vi "[ex ce] 1 Simplest client example.vi"() -> ()   [LabVIEW 2021]
doc: "<B>Simplest client example</B>\n\nThis example demonstrates simplest method to use CalcExpress for remote computation.\n\nTo execute this example, you need run <B>[ex ce] CE Server Example.vi</B> on either local or remote computer.\n\n::: CalcExpress Toolkit :::\nCopyright (c) 2000-2026 Konstantin Shifershteyn. All rights reserved."
uses:
  vi.lib/addons/CalcExpress/cetypes.llb/CalcExpress Data Type.ctl
panel:
  in  "Comment":string="To execute this example, you need run the \"[ex ce] CE Server Example.vi\" on either local or remote computer.\n---------------------------\nThis example demonstrates simplest method to use CalcExpress for remote computation.\n"
  in  "use TCP for local":bool
  in  "expression":string="/* initializes array of values in the range from -6*pi to 6*pi with step equal to 5 radians */\nx = nvecifs(-pi(6),pi(6), rad(5));\n\nsinc(x)  /* computes sin(x)/x */"
  out "graph":dbl[](graph)
  out "value type":T1=enum."DBL Number"
  out "error out":errorcluster
  in  "port":u32=3363
  in  "machine name (empty - localhost)":string
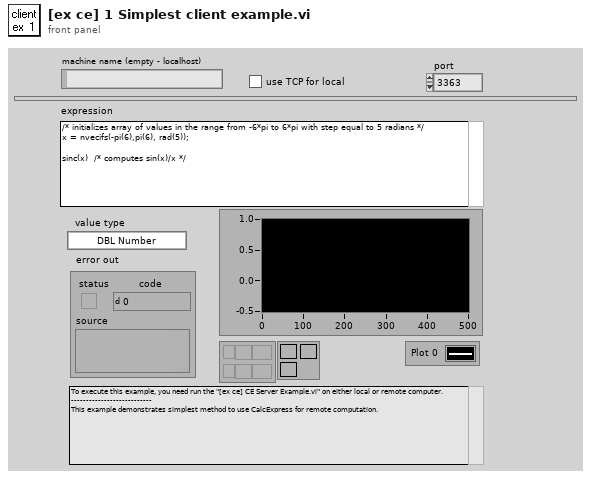
[diagram p1: front panel]
types:
  T1 = typedef "CalcExpress Data Type.ctl" = enum32{"String", "DBL Number", "identifier", "1D Array of DBL", "2D Array of DBL", "CDB Number", "1D Array of CDB", "2D Array of CDB", "1D Array of String", "2D Array of String", "Unknown data type"}
  T2 = typedef "CE Session.ctl" = cluster{"VI refnum":refnum<vi>, "VC Handle":T3}
  T3 = typedef "VarMan Variable Context Handle.ctl" = i32
  T4 = cluster{"type":T1, "dbl":dbl, "cdb":cdb, "str":string, "1d dbl":dbl[], "1d cdb":cdb[], "1d str":string[], "2d dbl":dbl[][], "2d cdb":cdb[][], "2d str":string[][]}
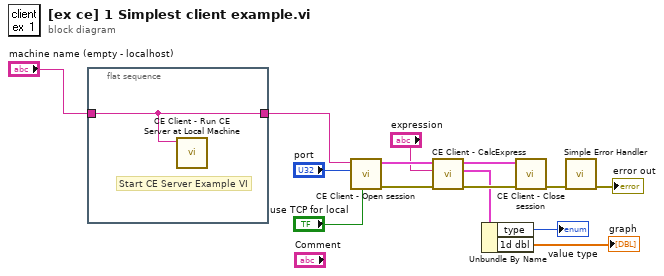
[diagram p0: block diagram]
diagram:
  n1 = flat-sequence {
    tunnel: [w15] -> w2
    tunnel: "machine name (empty - localhost)" -> [w15]
    frame #0 {
      # "Start CE Server Example VI"
      n2 = call "CE Client - Run CE Server at Local Machine.vi"("machine name"=w15) -> ()  [unwired: 9 in, 2 out]
    }
  }
  n3 = call "CE Client - Open session.vi"("use TCP for local (F)"="use TCP for local", "port number (3363)"="port", "machine name (empty - local)"=w2) -> ("error out"=w12:errorcluster, "CE session out"=w14:T2)  [unwired: 5 in]
  n4 = call "CE Client - CalcExpress.vi"("error in"=w12, "expression"="expression", "CE session"=w14) -> ("error out"=w11:errorcluster, "values out"=w4:T4, "dup CE session"=w13:T2)  [unwired: 4 in]
  n5 = Unbundle By Name(w4) -> ("type"=→"value type":T1, "1d dbl"=→"graph":dbl[])
  n6 = call "CE Client - Close session.vi"("error in"=w11, "CE session"=w13) -> ("error out"=w6:errorcluster)  [unwired: 6 in, 1 out]
  n7 = call <vilib>:"Simple Error Handler.vi"("error in (no error)"=w6) -> ("error out"=→"error out":errorcluster)  [unwired: 4 in, 4 out]
